vi "Read.vi"(8 "error in (no error)":errorcluster, 9 "timeout ms":i32, 10 "frames in":T1 {"flags" format="%.0x"; "id" format="%.0x"}, 11 "channel in":refnum<class "CANsub_Channel.lvclass">) -> (0 "error out":errorcluster, 2 "frames out":T1 {"flags" format="%.0x"; "id" format="%.0x"}, 3 "channel out":refnum<class "CANsub_Channel.lvclass">)   [LabVIEW 2021, in "CANsub_API.lvlib" / "CANsub_Channel.lvclass"]
doc: "Gives every frame that arrived since the last call, in the caller’s frames buffer (frames.count = number of frames). Waits at most timeout ms (0 = no wait). Answers pings by itself. On connection loss: state = Lost, error 5203. Must be overridden. Loop-safe: no allocation, bounded time."
uses:
  CANsub_Channel.lvclass
  Typedefs/CANsub_Frames.ctl
  CANsub_API.lvlib
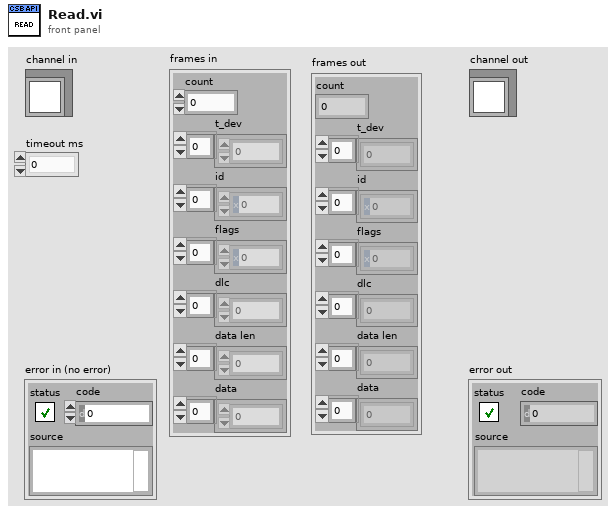
[diagram p1: front panel]
types:
  T1 = typedef "CANsub_API.lvlib/CANsub_Frames.ctl" = cluster{"count":i32, "t_dev":dbl[], "id":u32[], "flags":u16[], "dlc":u8[], "data len":u8[], "data":u8[]}
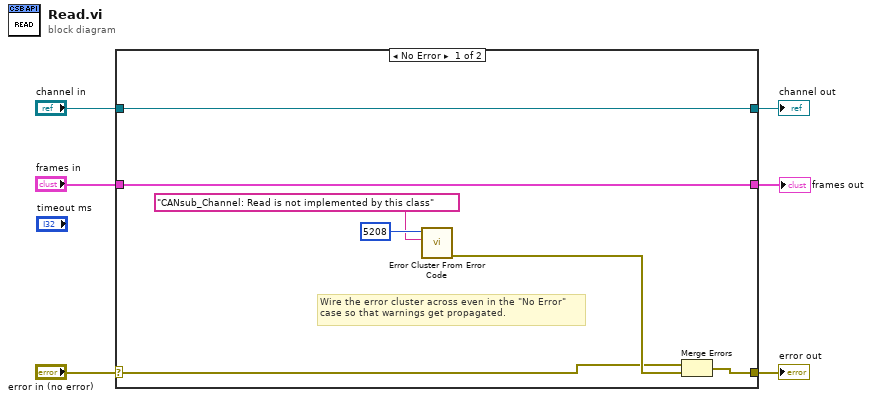
[diagram p0: block diagram]
diagram:
  n1 = case shown="No Error" "error in (no error)" {
    selector: "error in (no error)" -> [w7 w16]
    tunnel: [w8 w16] -> w5
    tunnel: [w13 w15] -> w3
    tunnel: "channel in" -> [w13 w15]
    tunnel: [w12 w14] -> w2
    tunnel: "frames in" -> [w12 w14]
    frame No Error {
      # "Wire the error cluster across even in the \"No Error\"\ncase so that warnings get propagated."
      n2 = call <vilib>:"Error Cluster From Error Code.vi"("error message (\"\")"="CANsub_Channel: Read is not implemented by this class" ("error message (\"\")"), "error code (0)"=5208) -> ("error out"=w11:errorcluster)  [unwired: 7 in]
      n3 = Merge Errors(w7, w11) -> (w8:errorcluster)
    }
    frame Error {
    }
  }
  "error out" <- w5
  "channel out" <- w3
  "frames out" <- w2
